vi "Shutoff SM.vi"(8 "error in (no error)":errorcluster, 11 "Puerto serial":refnum<visa-resource-name>) -> (0 "error out":errorcluster, 3 "Puerto serial":refnum<visa-resource-name>)   [LabVIEW 2020]
uses:
  5ac33253-7c67-463e-bba6-ac46ac7e0f6c.vi
  930877ef-ec65-47d0-bcaa-3321609e5bf5.vi
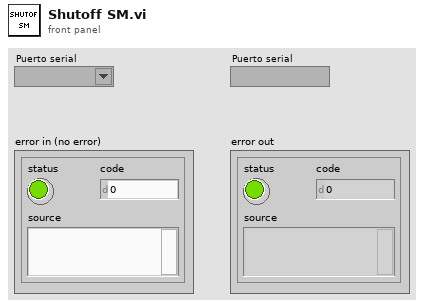
[diagram p1: front panel]
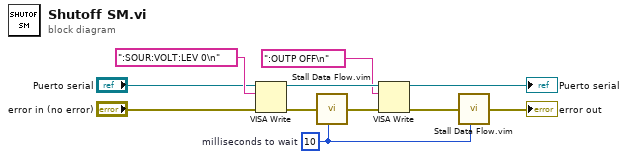
[diagram p0: block diagram]
diagram:
  w1 = u32 10  # milliseconds to wait
  n1 = VISA Write(VISA resource name="Puerto serial", write buffer=":SOUR:VOLT:LEV 0\n" ("Comando"), error in (no error)="error in (no error)") -> (VISA resource name out=w10:refnum<visa-resource-name>, error out=w11:errorcluster)  [unwired: 1 out]
  n2 = call "Stall Data Flow.vim"("value in"=w11, "milliseconds to wait"=w1) -> ("value out"=w3:errorcluster)  [unwired: 1 out]
  n3 = VISA Write(VISA resource name=w10, write buffer=":OUTP OFF\n" ("Comando"), error in (no error)=w3) -> (VISA resource name out=→"Puerto serial":refnum<visa-resource-name>, error out=w5:errorcluster)  [unwired: 1 out]
  n4 = call "Stall Data Flow.vim"("value in"=w5, "milliseconds to wait"=w1) -> ("value out"=→"error out":errorcluster)  [unwired: 1 out]
